vi "HOST_1712.vi"() -> ()   [LabVIEW 2018]
uses:
  <vilib>/userdefined/High Color/nirio_resource_hc.ctl
  <instrlib>/niDCPower/nidcpower.llb/niDCPower Measurement Type.ctl
  <vilib>/FPGAPlugInAG/PXI-7953R/niLvFpga_Open_PXI-7953R.vi
  <vilib>/rvi/interface/common/dynamic/niFpgaDynamicAddResources.vi
  <vilib>/FPGAPlugInAG/Dynamic/niLvFpga_Reset_Dynamic.vi
  <vilib>/FPGAPlugInAG/Dynamic/niLvFpga_Run_Dynamic.vi
  <vilib>/Utility/error.llb/Error Cluster From Error Code.vi
  <vilib>/rvi/errors/niLvFpgaAdjustHostInterfaceError.vi
  <vilib>/FPGAPlugInAG/Dynamic/niLvFpga_Close_Dynamic.vi
  <vilib>/rvi/interface/nirviOpenFPGA/nirviOpenFPGA.xnode
  FPGA Bitfiles/1712_FPGATarget_TARGET1712_pD+j9IKIark.lvbitx
  <vilib>/rvi/interface/nirviMethod/nirviMethod.xnode
  <vilib>/rvi/interface/nirviReadWriteControl/nirviReadWriteControl.xnode
  <vilib>/rvi/interface/nirviCloseFPGA/nirviCloseFPGA.xnode
  NiFpgaLv.dll
  <vilib>/rvi/interface/Simulation/niFpgaSimulationCallBeginRW.vi
  <vilib>/FPGAPlugInAG/Dynamic/niLvFpga_ReadFifo_Dynamic.vi
  <vilib>/rvi/errors/niLvFpgaMergeErrorWithErrorCode.vi
panel:
  in  "Tab Control":enum32{"Рабочая", "Служебная"}(tab)
  out "Image":T1(plugin-control)
  in  "Frames":path=path "D:/VPL/LabView/DOZOR_1712/DOZOR_1712/FRAMES"
  in  "LED":bool
  out "Номер образца":string="0"
  in  "Стоп":bool
  in  "Питание":bool
  in  "Линейки":bool
  in  "LOGS":path=path "D:/VPL/LabView/DOZOR_1712/DOZOR_1712/LOGS"
  in  "resource name":T2="PXI1Slot6"
  in  "1":refnum<k15>="PXI1Slot3" caption="instrument handle"
  in  "0":refnum<k15>="PXI1Slot2" caption="instrument handle"
  in  "2":refnum<k15>="PXI1Slot4" caption="instrument handle"
  in  "-15, V":dbl=-15.0 caption="voltage level" format="%_6p"
  out "-15_cur":dbl caption="measurement" format="%_6g"
  in  "-15_curlim":dbl=0.1 caption="current limit" format="%_6p"
  out "4V_cur":dbl caption="measurement" format="%_6g"
  in  "4V_curlim":dbl=0.15 caption="current limit" format="%_6p"
  in  "4V":dbl=4.0 caption="voltage level" format="%_6p"
  in  "1V":dbl=1.0 caption="voltage level" format="%_6p"
  in  "STAB, V":dbl=10.0 caption="voltage level" format="%_6p"
  out "VDD_cur":dbl caption="measurement" format="%_6g"
  out "1V_cur":dbl caption="measurement" format="%_6g"
  out "PH_LOW_cur":dbl caption="measurement" format="%_6g"
  out "RD_cur":dbl caption="measurement" format="%_6g"
  out "STAB_cur":dbl caption="measurement" format="%_6g"
  out "ADC_cur":dbl caption="measurement" format="%_6g"
  in  "VDD_curlim":dbl=0.15 caption="current limit" format="%_6p"
  in  "1V_curlim":dbl=0.01 caption="current limit" format="%_6p"
  in  "PH_LOW_curlim":dbl=0.3 caption="current limit" format="%_6p"
  in  "RD_curlim":dbl=0.1 caption="current limit" format="%_6p"
  in  "STAB_curlim":dbl=0.2 caption="current limit" format="%_6p"
  in  "ADC_curlim":dbl=0.2 caption="current limit" format="%_6p"
  in  "VDD, V":dbl=17.0 caption="voltage level" format="%_6p"
  in  "PH_LOW, V":dbl=-3.5 caption="voltage level" format="%_6p"
  in  "RD, V":dbl=13.1 caption="voltage level" format="%_6p"
  in  "ADC, V":dbl=6.0 caption="voltage level" format="%_6p"
  out "PS_LOW_cur":dbl caption="measurement" format="%_6g"
  in  "PS_LOW_curlim":dbl=0.1 caption="current limit" format="%_6p"
  in  "PS_LOW, V":dbl=-8.0 caption="voltage level" format="%_6p"
  out "ADC":bool
  out "4V":bool
  out "1V":bool
  out "1V":i32
  out "PH":i32
  out "RD":i32
  out "4V":i32
  out "-15":i32
  out "STAB":i32
  out "ADC":i32
  out "PS":i32
  out "VDD":i32
  in  "4V_selcur":dbl=0.025 caption="current limit" format="%_6p"
  in  "RD_selcur":dbl=0.01 caption="current limit" format="%_6p"
  in  "PH_LOW_selcur":dbl=0.025 caption="current limit" format="%_6p"
  in  "ADC_selcur":dbl=0.15 caption="current limit" format="%_6p"
  in  "STAB_selcur":dbl=0.1 caption="current limit" format="%_6p"
  in  "-15_selcur":dbl=0.009999999999999998 caption="current limit" format="%_6p"
  in  "1V_selcur":dbl=0.01 caption="current limit" format="%_6p"
  in  "VDD_selcur":dbl=0.075 caption="current limit" format="%_6p"
  in  "PS_LOW_selcur":dbl=0.01 caption="current limit" format="%_6p"
  out "STAB":bool
  out "-15":bool
  out "RD":bool
  out "PH":bool
  out "VDD":bool
  out "PS":bool
  in  "Какая фотка?":string
  in  "ПРИМЕЧАНИЕ":string
  out "СКО":dbl
  out "Среднее":dbl
  in  "Запись Кадра":bool
  out "FRAME_OK":bool
  in  "2/4 V":enum16{"2V", "4V"}(ring)
  in  "3CH/1CH":enum16{"3CH", "1CH"}(ring)=enum."1CH"
  out "Configuration":bool[](array[boolean])
  in  "Какой канал?":enum16{"OUT1", "OUT2", "OUT3"}(ring)
  in  "Прошить АЦП":bool
  out "АЦП прошит!":bool
  in  "НЕПРЕРЫВНО":bool
  in  "文韧 世男!":bool
  in  "ПЕРЕБОР?":bool
  out "Канал":string="1"
  in  "SIM_SEL":bool
  out "SEL":bool
  out "FRAME":u16[][](array[numeric])
  out "OUT":cluster{u16, u16, u16, u16}[][](array[cluster])
  in  "Сколько строк?":i32=270
  in  "1163":u16=1163
  in  "PS1_2":u16=980
  in  "PS1_1":u16=300
  in  "PS21_1":u16=165
  in  "PS21_2":u16=573
  in  "PS3_1":u16=435
  in  "PS3_2":u16=843
  in  "PS41_1":u16=30
  in  "PS41_2":u16=710
  in  "CDS1_2":u8=14
  in  "CDS1_1":u8=9
  in  "CDS2_2":u8=18
  in  "CDS2_1":u8=5
  in  "ADC_2":u8=22
  in  "ADC_1":u8=9
  in  "RG_2":u8=8
  in  "RG1":u8=5
  in  "PH2_2":u8=17
  in  "PH2_1":u8=5
  in  "PH1_2":u8=17
  in  "PH1_1":u8=5
  in  "HOR":u16=465
  in  "8":u8=24
  in  "LOW":u8=9
  in  "HIGH":u8=22
  in  "Усреднение":i32=1
  in  "Между кадрами, мс":u8=1
  in  "ISO":dbl=1.0
  in  "+/- OUT2":enum16{"-", "+"}(ring)=enum."+"
  in  "Смещение, до 300_OUT2":dbl
  in  "Усиление (до 6)_OUT2":u8=1
  in  "Усиление (до 6)_OUT4":u8=1
  in  "+/- OUT4":enum16{"-", "+"}(ring)=enum."+"
  in  "Смещение, до 300_OUT4":dbl
  in  "Усиление (до 6)_OUT1":u8=1
  in  "Смещение, до 300_OUT1":dbl
  in  "+/- OUT1":enum16{"-", "+"}(ring)=enum."+"
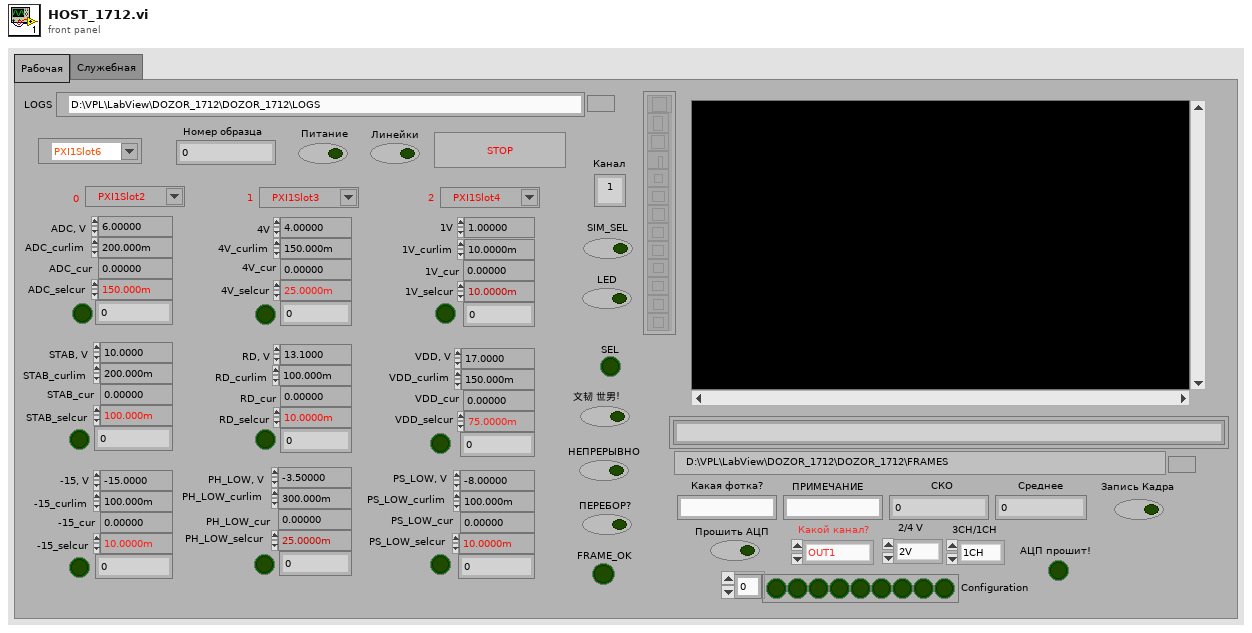
[diagram p1: front panel]
types:
  T1 = typedef "IMAQ Image.ctl" = refnum<image>
  T2 = typedef "nirio_resource_hc.ctl" = tag
  T3 = enum16{"open", "replace", "create", "open or create", "replace or create", "replace or create with confirmation"}
  T4 = typedef "niDCPower Measurement Type.ctl" = i32
  T5 = typedef "Image Type" = u32
  T6 = enum16{"Configuration", "MUX", "RED PGA", "GREEN PGA", "BLUE PGA", "RED OFF", "GREEN OFF", "BLUE OFF"}
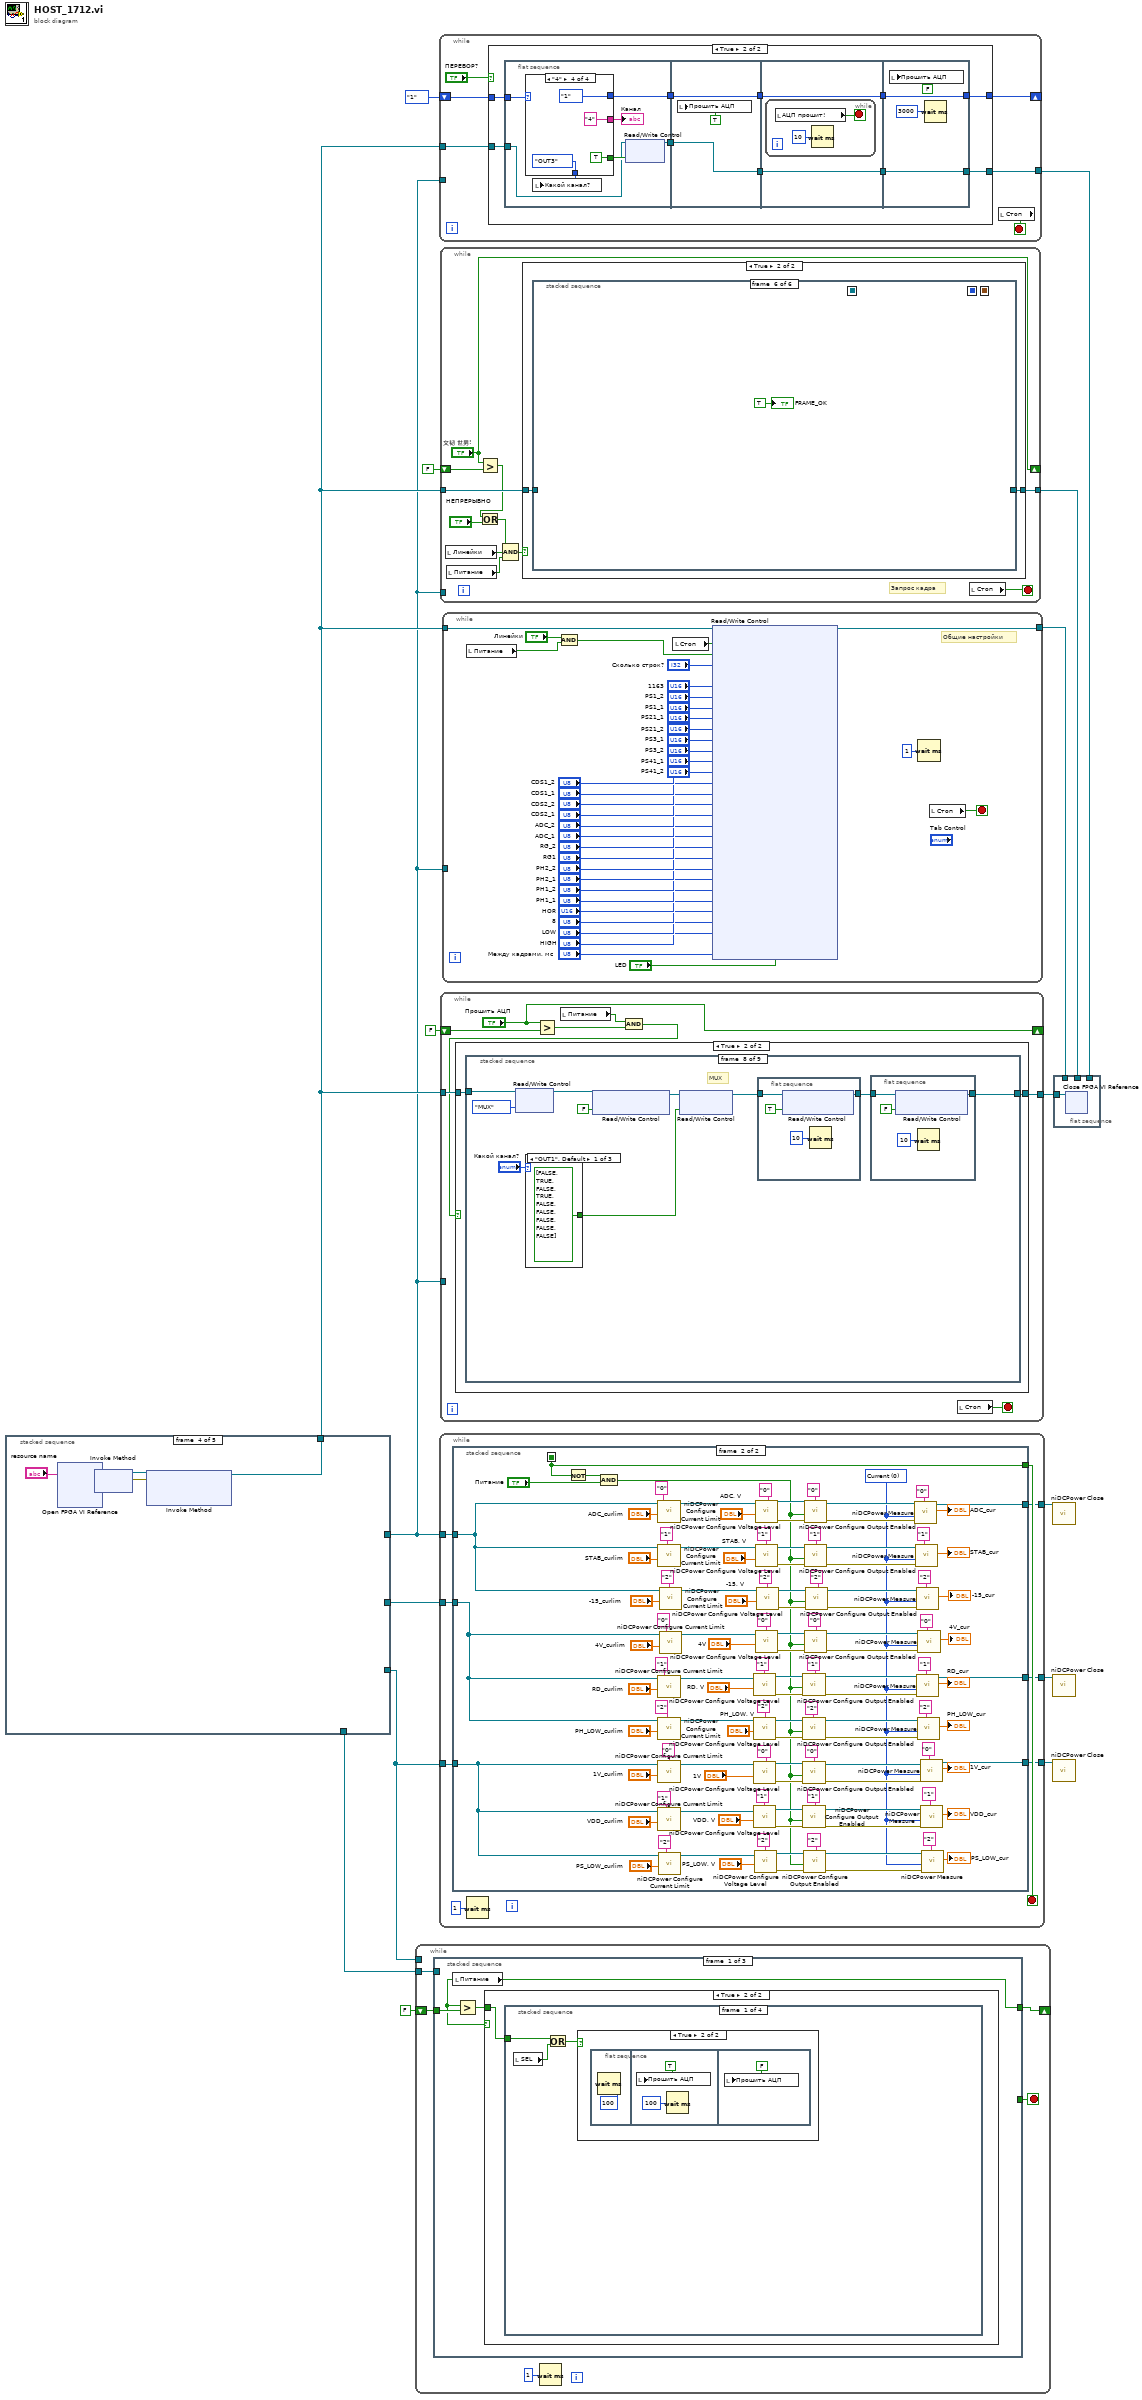
[diagram p0: block diagram]
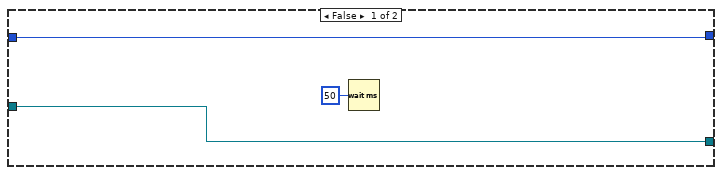
[diagram p2: hidden frame]
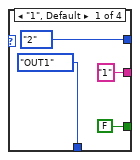
[diagram p3: hidden frame]
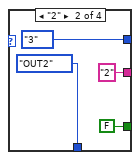
[diagram p4: hidden frame]
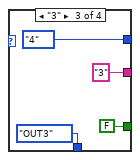
[diagram p5: hidden frame]
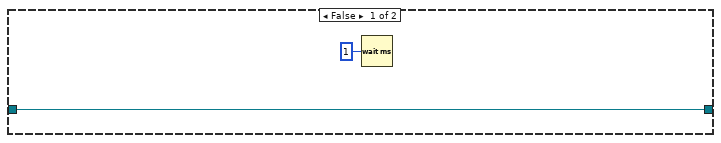
[diagram p6: hidden frame]
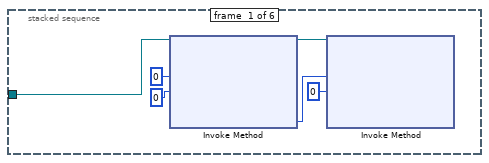
[diagram p7: hidden frame]
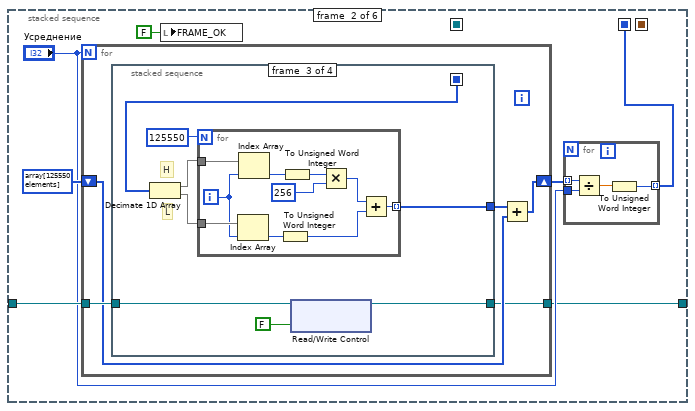
[diagram p8: hidden frame]
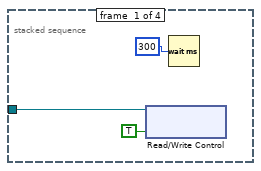
[diagram p9: hidden frame]
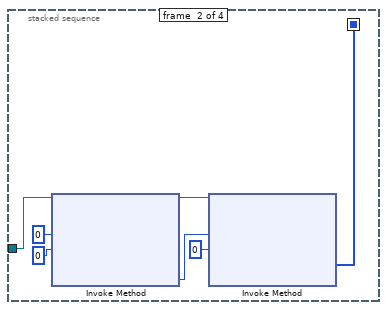
[diagram p10: hidden frame]
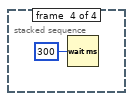
[diagram p11: hidden frame]
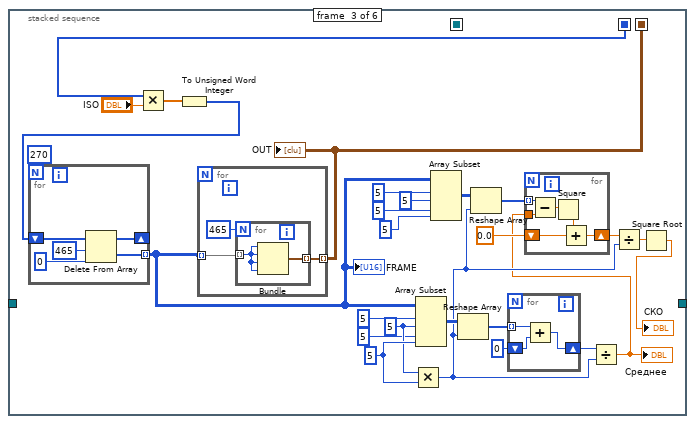
[diagram p12: hidden frame]
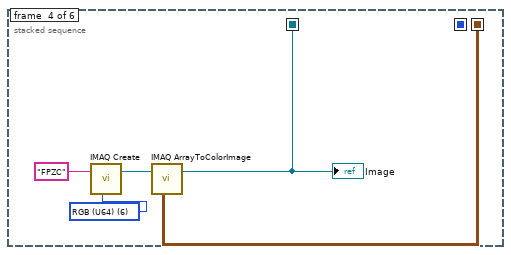
[diagram p13: hidden frame]
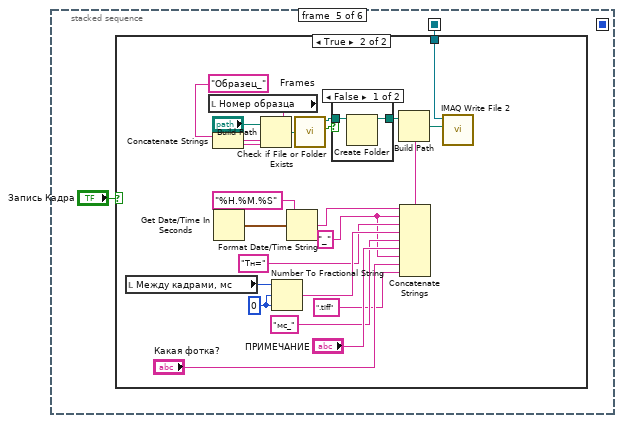
[diagram p14: hidden frame]
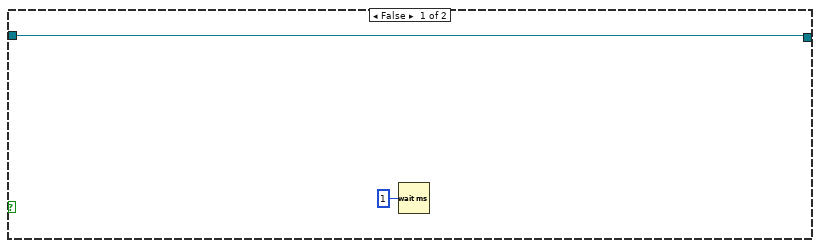
[diagram p17: hidden frame]
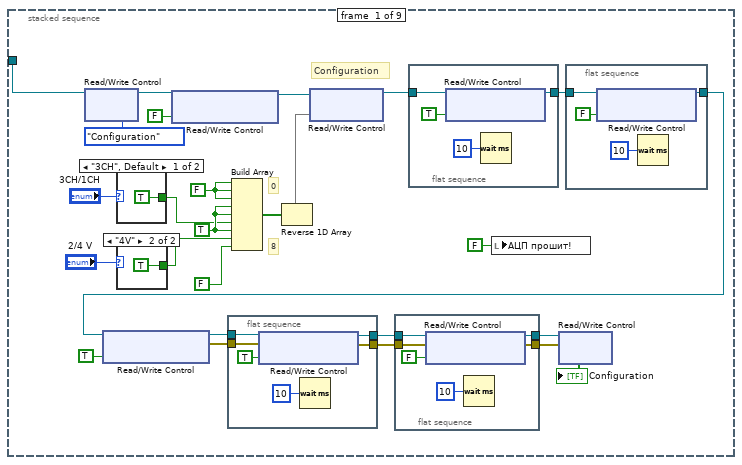
[diagram p18: hidden frame]
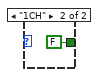
[diagram p19: hidden frame]
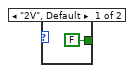
[diagram p20: hidden frame]
diagram:
  n1 = stacked-sequence {
    tunnel: [_ _ _ _ w67] -> w6
    tunnel: [_ _ _ _ w66] -> w9
    tunnel: [_ _ _ _ w65] -> w16
    tunnel: [_ _ _ w59 _] -> w10
    tunnel: [_ _ w22 _ _] -> w11
    frame #0 {
      n2 = call "Begin.vi"() -> ("Номер образца 2"=→"Номер образца":string)  [unwired: 11 in]
    }
    frame #1 {
      w18 = FALSE
      w20 = 0 ("VDD")
      w19 = "" ("Какая фотка?")
      # "Отжатие кнопок, обнуление счетчиков"
      n3 = local write "Какой канал?"(enum16{"OUT1", "OUT2", "OUT3"}."OUT1" ("Какой канал?")) -> ()
      n4 = local write "Запись Кадра"(w18) -> ()
      n5 = local write "НЕПРЕРЫВНО"(w18) -> ()
      n6 = local write "ПЕРЕБОР?"(w18) -> ()
      n7 = local write "FRAME_OK"(w18) -> ()
      n8 = local write "Прошить АЦП"(w18) -> ()
      n9 = local write "文韧 世男!"(w18) -> ()
      n10 = local write "АЦП прошит!"(w18) -> ()
      n11 = local write "SIM_SEL"(w18) -> ()
      n12 = local write "Стоп"(w18) -> ()
      n13 = local write "Питание"(w18) -> ()
      n14 = local write "Линейки"(w18) -> ()
      n15 = local write "LED"(w18) -> ()
      n16 = local write "Какая фотка?"(w19) -> ()
      n17 = local write "ПРИМЕЧАНИЕ"(w19) -> ()
      n18 = local write "VDD"(w20) -> ()
      n19 = local write "RD"(w20) -> ()
      n20 = local write "PH"(w20) -> ()
      n21 = local write "PS"(w20) -> ()
      n22 = local write "1V"(w20) -> ()
      n23 = local write "ADC"(w20) -> ()
      n24 = local write "STAB"(w20) -> ()
      n25 = local write "-15"(w20) -> ()
      n26 = local write "4V"(w20) -> ()
    }
    frame #2 {
      w24 = "\t"
      n27 = local read "Номер образца"() -> (w51:string)
      n28 = Build Path(base path="LOGS", name or relative path=w51) -> (appended path=w48:path)
      n29 = Get Date/Time In Seconds() -> (seconds since 1Jan1904=w45:timestamp)
      n30 = call <vilib>:"Check if File or Folder Exists.vi"("path"=w48) -> ("file or folder exists?"=w49:bool, "dup path"=w50:path)  [unwired: 8 in, 1 out]
      n31 = Format Date/Time String(time format string (%c)="%d %H.%M.%S", seconds (now)=w45) -> (date/time string=w43:string)  [unwired: 1 in]
      n32 = case shown="False" w49 {
        tunnel: w50 -> [w57 w58]
        tunnel: [w56 w58] -> w40
        frame False {
          n33 = Create Folder(path (use dialog)=w57) -> (created path=w56:path)  [unwired: 2 in, 2 out]
        }
        frame True {
        }
      }
      n34 = Concatenate Strings(w43, ".xls" ("string")) -> (w42:string)
      n35 = Build Path(base path=w40, name or relative path=w42) -> (appended path=w44:path)
      n36 = Open/Create/Replace File(file path (use dialog)=w44, operation (0:open)=T3."open or create", access (0:read/write)=enum16{"read/write", "read-only", "write-only"}."read/write") -> (refnum out=w46:refnum<file>)  [unwired: 3 in, 2 out]
      n37 = case shown="True" TRUE {
        tunnel: w46 -> [w52 w55]
        tunnel: [w52 w53] -> w41
        frame False {
        }
        frame True {
          n38 = Set File Position(refnum=w55, from (0:start)=enum16{"start", "end", "current"}."end") -> (refnum out=w53:refnum<file>)  [unwired: 2 in, 1 out]
        }
      }
      n39 = Format Into String(initial string=w41, "Time" ("input 1"), w24, "ADC_cur", w24, "STAB_cur", w24, "-15_cur", w24, "4_cur", w24, "RD_cur", w24, "PH_LOW_cur", w24, "1V_cur", w24, "VDD_cur", w24, "PS_LOW_cur", "\r\n") -> (resulting string=w22:refnum<file>)  [unwired: 2 in, 1 out]
    }
    frame #3 {
      n40 = xnode "Open FPGA VI Reference"("resource name"="resource name") -> ("FPGA VI Reference Out"=w60:refnum<k20>, "error out"=w62:errorcluster)  [unwired: 1 in]
      n41 = xnode "Invoke Method"("FPGA VI Reference In"=w60, "error in"=w62) -> ("FPGA VI Reference Out"=w63:refnum<k20>, "error out"=w61:errorcluster)
      n42 = xnode "Invoke Method"("FPGA VI Reference In"=w63, "error in"=w61) -> ("FPGA VI Reference Out"=w59:refnum<k20>)  [unwired: 1 in, 1 out]
    }
    frame #4 {
      n43 = call <instrlib>:"niDCPower Initialize.vi"("resource name"="2") -> ("error out"=w73:errorcluster, "instrument handle out"=w70:refnum<k15>)  [unwired: 3 in, 6 out]
      n44 = call <instrlib>:"niDCPower Initialize.vi"("resource name"="1") -> ("error out"=w71:errorcluster, "instrument handle out"=w68:refnum<k15>)  [unwired: 3 in, 6 out]
      n45 = call <instrlib>:"niDCPower Initialize.vi"("resource name"="0") -> ("error out"=w72:errorcluster, "instrument handle out"=w69:refnum<k15>)  [unwired: 3 in, 6 out]
      n46 = call <instrlib>:"niDCPower Configure Voltage Level.vi"("error in (no error)"=w73, "voltage level"=0.0, "channel name"="0,1,2", "instrument handle"=w70) -> ("instrument handle out"=w67:refnum<k15>)  [unwired: 6 in, 1 out]
      n47 = call <instrlib>:"niDCPower Configure Voltage Level.vi"("error in (no error)"=w71, "voltage level"=0.0, "channel name"="0,1,2", "instrument handle"=w68) -> ("instrument handle out"=w65:refnum<k15>)  [unwired: 6 in, 1 out]
      n48 = call <instrlib>:"niDCPower Configure Voltage Level.vi"("error in (no error)"=w72, "voltage level"=0.0, "channel name"="0,1,2", "instrument handle"=w69) -> ("instrument handle out"=w66:refnum<k15>)  [unwired: 6 in, 1 out]
    }
  }
  n49 = while {
    tunnel: w11 -> [w85]
    shift-right: [w83] -> _
    shift-left: FALSE -> [w84]
    tunnel: w6 -> [_]
    stop <- w86 stop-if-true
    n50 = stacked-sequence {
      tunnel: [_ _ w227] -> w86
      tunnel: w85 -> [_ w203 _]
      tunnel: w84 -> [w90 _ _]
      tunnel: [w88 _ _] -> w83
      frame #0 {
        n51 = local read "Питание"() -> (w88:bool)
        n52 = Greater?(x=w88, y=w90) -> (0:w89:bool)
        n53 = case shown="True" w88 {
          tunnel: w89 -> [_ w91]
          frame False {
          }
          frame True {
            n54 = stacked-sequence {
              tunnel: w91 -> [w93 _ _ _]
              frame #0 {
                n55 = local read "SEL"() -> (w92:bool)
                n56 = Or(x=w93, y=w92) -> (x .or. y?=w94:bool)
                n57 = case shown="True" w94 {
                  frame False {
                  }
                  frame True {
                    n58 = flat-sequence {
                      frame #0 {
                        n59 = Wait (ms)(milliseconds to wait=u32 100) -> ()  [unwired: 1 out]
                      }
                      frame #1 {
                        n60 = local write "Прошить АЦП"(TRUE ("Прошить АЦП")) -> ()
                        n61 = Wait (ms)(milliseconds to wait=u32 100) -> ()  [unwired: 1 out]
                      }
                      frame #2 {
                        n62 = local write "Прошить АЦП"(FALSE ("Прошить АЦП")) -> ()
                      }
                    }
                  }
                }
              }
              frame #1 {
                n63 = local read "PH_LOW_cur"() -> (w121:dbl)
                n64 = local read "PS_LOW_cur"() -> (w124:dbl)
                n65 = local read "STAB_cur"() -> (w100:dbl)
                n66 = local read "ADC_cur"() -> (w109:dbl)
                n67 = local read "VDD_cur"() -> (w106:dbl)
                n68 = local read "-15_cur"() -> (w118:dbl)
                n69 = local read "RD_cur"() -> (w103:dbl)
                n70 = local read "4V_cur"() -> (w112:dbl)
                n71 = local read "1V_cur"() -> (w115:dbl)
                n72 = Greater?(x=w100, y="STAB_selcur") -> (0:→"STAB":bool)
                n73 = Greater?(x=w103, y="RD_selcur") -> (0:→"RD":bool)
                n74 = Greater?(x=w106, y="VDD_selcur") -> (0:→"VDD":bool)
                n75 = Greater?(x=w109, y="ADC_selcur") -> (0:→"ADC":bool)
                n76 = Greater?(x=w112, y="4V_selcur") -> (0:→"4V":bool)
                n77 = Greater?(x=w115, y="1V_selcur") -> (0:→"1V":bool)
                n78 = Greater?(x=w118, y="-15_selcur") -> (0:→"-15":bool)
                n79 = Greater?(x=w121, y="PH_LOW_selcur") -> (0:→"PH":bool)
                n80 = Greater?(x=w124, y="PS_LOW_selcur") -> (0:→"PS":bool)
              }
              frame #2 {
                n81 = local read "ADC"() -> (w132:bool)
                n82 = local read "STAB"() -> (w133:bool)
                n83 = local read "-15"() -> (w134:bool)
                n84 = local read "4V"() -> (w129:bool)
                n85 = local read "VDD"() -> (w130:bool)
                n86 = local read "PS"() -> (w131:bool)
                n87 = case shown="True" w130 {
                  frame False {
                  }
                  frame True {
                    n88 = local read "VDD"() -> (w152:i32)
                    n89 = Increment(x=w152) -> (x+1=→"VDD":i32)
                  }
                }
                n90 = case shown="True" w131 {
                  frame False {
                  }
                  frame True {
                    n91 = local read "PS"() -> (w150:i32)
                    n92 = Increment(x=w150) -> (x+1=→"PS":i32)
                  }
                }
                n93 = case shown="True" w132 {
                  frame False {
                  }
                  frame True {
                    n94 = local read "ADC"() -> (w148:i32)
                    n95 = Increment(x=w148) -> (x+1=→"ADC":i32)
                  }
                }
                n96 = case shown="True" w133 {
                  frame False {
                  }
                  frame True {
                    n97 = local read "STAB"() -> (w146:i32)
                    n98 = Increment(x=w146) -> (x+1=→"STAB":i32)
                  }
                }
                n99 = case shown="True" w134 {
                  frame False {
                  }
                  frame True {
                    n100 = local read "-15"() -> (w144:i32)
                    n101 = Increment(x=w144) -> (x+1=→"-15":i32)
                  }
                }
                n102 = case shown="True" w129 {
                  frame False {
                  }
                  frame True {
                    n103 = local read "4V"() -> (w142:i32)
                    n104 = Increment(x=w142) -> (x+1=→"4V":i32)
                  }
                }
                n105 = local read "RD"() -> (w128:bool)
                n106 = local read "PH"() -> (w127:bool)
                n107 = local read "1V"() -> (w126:bool)
                n108 = case shown="True" w127 {
                  frame False {
                  }
                  frame True {
                    n109 = local read "PH"() -> (w138:i32)
                    n110 = Increment(x=w138) -> (x+1=→"PH":i32)
                  }
                }
                n111 = case shown="True" w128 {
                  frame False {
                  }
                  frame True {
                    n112 = local read "RD"() -> (w140:i32)
                    n113 = Increment(x=w140) -> (x+1=→"RD":i32)
                  }
                }
                n114 = case shown="True" w126 {
                  frame False {
                  }
                  frame True {
                    n115 = local read "1V"() -> (w136:i32)
                    n116 = Increment(x=w136) -> (x+1=→"1V":i32)
                  }
                }
              }
              frame #3 {
                n117 = local read "STAB"() -> (w163:bool)
                n118 = local read "ADC"() -> (w164:bool)
                n119 = local read "VDD"() -> (w166:bool)
                n120 = local read "-15"() -> (w162:bool)
                n121 = local read "PH"() -> (w159:bool)
                n122 = local read "RD"() -> (w160:bool)
                n123 = local read "PS"() -> (w165:bool)
                n124 = local read "4V"() -> (w161:bool)
                n125 = local read "1V"() -> (w158:bool)
                n126 = Compound Arithmetic op=OR(w166, w165, w164, w163, w162, w161, w160, w159, w158) -> (w154:bool)
                n127 = local read "Линейки"() -> (w156:bool)
                n128 = local read "Питание"() -> (w157:bool)
                n129 = Or(x=w154, y="SIM_SEL") -> (x .or. y?=w153:bool)
                "SEL" <- w153
                n130 = case shown="True" w153 {
                  tunnel: w156 -> [_ w173]
                  tunnel: w157 -> [_ w172]
                  frame False {
                    n131 = Wait (ms)(milliseconds to wait=u32 1) -> ()  [unwired: 1 out]
                  }
                  frame True {
                    n132 = flat-sequence {
                      tunnel: w173 -> [w175]
                      tunnel: w172 -> [w174]
                      tunnel: [w175] -> w170
                      tunnel: [w174] -> w169
                      tunnel: [w178] -> w171
                      tunnel: w170 -> [w178]
                      tunnel: w169 -> [w177]
                      tunnel: [w177] -> w168
                      tunnel: w171 -> [w181]
                      tunnel: w168 -> [w180]
                      frame #0 {
                        w176 = FALSE ("Питание")
                        n133 = local write "Питание"(w176) -> ()
                        n134 = local write "Линейки"(w176) -> ()
                      }
                      frame #1 {
                        n135 = Wait (ms)(milliseconds to wait=u32 100) -> ()  [unwired: 1 out]
                      }
                      frame #2 {
                        n136 = local write "Линейки"(w181) -> ()
                        n137 = local write "Питание"(w180) -> ()
                      }
                    }
                  }
                }
              }
            }
          }
        }
      }
      frame #1 {
        w202 = i16 0 ("width (-)")
        w205 = i16 3 ("width (-)")
        w201 = "\t"
        # "Логирование данных"
        n138 = local read "STAB"() -> (w189:i32)
        n139 = local read "ADC"() -> (w190:i32)
        n140 = local read "VDD"() -> (w183:i32)
        n141 = local read "-15"() -> (w188:i32)
        n142 = local read "PH"() -> (w185:i32)
        n143 = local read "RD"() -> (w186:i32)
        n144 = local read "4V"() -> (w187:i32)
        n145 = local read "1V"() -> (w184:i32)
        n146 = local read "PS"() -> (w182:i32)
        n147 = Number To Fractional String(number=w190, width (-)=w202, precision (6)=w202) -> (F-format string=w199:string)  [unwired: 1 in]
        n148 = Number To Fractional String(number=w189, width (-)=w202, precision (6)=w202) -> (F-format string=w198:string)  [unwired: 1 in]
        n149 = Number To Fractional String(number=w188, width (-)=w202, precision (6)=w202) -> (F-format string=w197:string)  [unwired: 1 in]
        n150 = Number To Fractional String(number=w187, width (-)=w202, precision (6)=w202) -> (F-format string=w196:string)  [unwired: 1 in]
        n151 = Number To Fractional String(number=w186, width (-)=w202, precision (6)=w202) -> (F-format string=w195:string)  [unwired: 1 in]
        n152 = Number To Fractional String(number=w185, width (-)=w202, precision (6)=w202) -> (F-format string=w194:string)  [unwired: 1 in]
        n153 = Number To Fractional String(number=w184, width (-)=w202, precision (6)=w202) -> (F-format string=w193:string)  [unwired: 1 in]
        n154 = Number To Fractional String(number=w183, width (-)=w202, precision (6)=w202) -> (F-format string=w192:string)  [unwired: 1 in]
        n155 = Number To Fractional String(number=w182, width (-)=w202, precision (6)=w202) -> (F-format string=w191:string)  [unwired: 1 in]
        n156 = local read "PH_LOW_cur"() -> (w209:dbl)
        n157 = local read "PS_LOW_cur"() -> (w206:dbl)
        n158 = local read "STAB_cur"() -> (w213:dbl)
        n159 = local read "ADC_cur"() -> (w214:dbl)
        n160 = local read "VDD_cur"() -> (w207:dbl)
        n161 = local read "-15_cur"() -> (w212:dbl)
        n162 = local read "RD_cur"() -> (w210:dbl)
        n163 = local read "4V_cur"() -> (w211:dbl)
        n164 = local read "1V_cur"() -> (w208:dbl)
        n165 = Number To Fractional String(number=w214, width (-)=w205, precision (6)=w205) -> (F-format string=w223:string)  [unwired: 1 in]
        n166 = Number To Fractional String(number=w213, width (-)=w205, precision (6)=w205) -> (F-format string=w222:string)  [unwired: 1 in]
        n167 = Number To Fractional String(number=w212, width (-)=w205, precision (6)=w205) -> (F-format string=w221:string)  [unwired: 1 in]
        n168 = Number To Fractional String(number=w211, width (-)=w205, precision (6)=w205) -> (F-format string=w220:string)  [unwired: 1 in]
        n169 = Number To Fractional String(number=w210, width (-)=w205, precision (6)=w205) -> (F-format string=w219:string)  [unwired: 1 in]
        n170 = Number To Fractional String(number=w209, width (-)=w205, precision (6)=w205) -> (F-format string=w218:string)  [unwired: 1 in]
        n171 = Number To Fractional String(number=w208, width (-)=w205, precision (6)=w205) -> (F-format string=w217:string)  [unwired: 1 in]
        n172 = Number To Fractional String(number=w207, width (-)=w205, precision (6)=w205) -> (F-format string=w216:string)  [unwired: 1 in]
        n173 = Number To Fractional String(number=w206, width (-)=w205, precision (6)=w205) -> (F-format string=w215:string)  [unwired: 1 in]
        n174 = Get Date/Time In Seconds() -> (seconds since 1Jan1904=w226:timestamp)
        n175 = Format Date/Time String(time format string (%c)="%d %H:%M:%S:%3u", seconds (now)=w226) -> (date/time string=w224:string)  [unwired: 1 in]
        n176 = Concatenate Strings(w224, w201, w223, w201, w222, w201, w221, w201, w220, w201, w219, w201, w218, w201, w217, w201, w216, w201, w215, w201, w199, w201, w198, w201, w197, w201, w196, w201, w195, w201, w194, w201, w193, w201, w192, w201, w191, "\r\n") -> (w225:string)
        n177 = Format Into String(initial string=w203, w225) -> ()  [unwired: 2 in, 2 out]
      }
      frame #2 {
        n178 = local read "Стоп"() -> (w227:bool)
      }
    }
    n179 = Wait (ms)(milliseconds to wait=u32 1) -> ()  [unwired: 1 out]
  }
  n180 = while {
    tunnel: w10 -> [w231]
    tunnel: w9 -> [_]
    shift-right: [w229] -> _
    shift-left: enum16{"1", "2", "3", "4"}."1" -> [w230]
    tunnel: [w228] -> w1
    stop <- w233 stop-if-true
    n181 = case shown="True" "ПЕРЕБОР?" {
      tunnel: w231 -> [w234 w246]
      tunnel: w230 -> [w235 w245]
      tunnel: [w235 w241] -> w229
      tunnel: [w234 w240] -> w228
      frame False {
        n182 = Wait (ms)(milliseconds to wait=u32 50) -> ()  [unwired: 1 out]
      }
      frame True {
        n183 = flat-sequence {
          tunnel: w246 -> [w249]
          tunnel: w245 -> [w253]
          tunnel: [w252] -> w244
          tunnel: [w247] -> w237
          tunnel: w244 -> [w271]
          tunnel: [w271] -> w242
          tunnel: [w270] -> w238
          tunnel: w237 -> [w270]
          tunnel: [w274] -> w243
          tunnel: w242 -> [w274]
          tunnel: [w273] -> w239
          tunnel: w238 -> [w273]
          tunnel: w243 -> [w278]
          tunnel: [w278] -> w241
          tunnel: [w277] -> w240
          tunnel: w239 -> [w277]
          frame #0 {
            n184 = case shown="\"4\"" w253 {
              tunnel: [enum16{"1", "2", "3", "4"}."2" enum16{"1", "2", "3", "4"}."3" enum16{"1", "2", "3", "4"}."4" enum16{"1", "2", "3", "4"}."1"] -> w252
              tunnel: [FALSE ("VNR") FALSE ("VNR") FALSE ("VNR") TRUE ("VNR")] -> w251
              tunnel: ["1" "2" "3" "4"] -> w250
              tunnel: [enum16{"OUT1", "OUT2", "OUT3"}."OUT1" ("Какой канал?") enum16{"OUT1", "OUT2", "OUT3"}."OUT2" ("Какой канал?") enum16{"OUT1", "OUT2", "OUT3"}."OUT3" ("Какой канал?") enum16{"OUT1", "OUT2", "OUT3"}."OUT3" ("Какой канал?")] -> w248
              frame "1", Default {
              }
              frame "2" {
              }
              frame "3" {
              }
              frame "4" {
              }
            }
            "Канал" <- w250
            n185 = local write "Какой канал?"(w248) -> ()
            n186 = xnode "Read/Write Control"("FPGA VI Reference In"=w249, "VNR"=w251) -> ("FPGA VI Reference Out"=w247:refnum<k20>)  [unwired: 1 in, 1 out]
          }
          frame #1 {
            n187 = local write "Прошить АЦП"(TRUE ("Прошить АЦП")) -> ()
          }
          frame #2 {
            n188 = while {
              stop <- w276 stop-if-true
              n189 = local read "АЦП прошит!"() -> (w276:bool)
              n190 = Wait (ms)(milliseconds to wait=u32 10) -> ()  [unwired: 1 out]
            }
          }
          frame #3 {
            n191 = local write "Прошить АЦП"(FALSE ("Прошить АЦП")) -> ()
            n192 = Wait (ms)(milliseconds to wait=u32 3000) -> ()  [unwired: 1 out]
          }
        }
      }
    }
    n193 = local read "Стоп"() -> (w233:bool)
  }
  n194 = while {
    tunnel: w9 -> [w287]
    tunnel: w16 -> [w286]
    tunnel: w6 -> [w285]
    tunnel: [w283] -> w15
    tunnel: [w282] -> w14
    tunnel: [w281] -> w13
    stop <- w284 stop-if-true
    n195 = stacked-sequence {
      seq-local: ["Стоп" _] -> [_ w290]
      tunnel: w285 -> [_ w295]
      tunnel: [_ w336] -> w283
      tunnel: [_ w335] -> w282
      tunnel: [_ w334] -> w281
      tunnel: w287 -> [_ w294]
      tunnel: w286 -> [_ w293]
      tunnel: [_ w290] -> w284
      frame #0 {
      }
      frame #1 {
        w296 = T4 0 items=["Current", "Voltage"] ("measurement type")
        n196 = Not(x=w290) -> (.not. x?=w309:bool)
        n197 = And(x=w309, y="Питание") -> (x .and. y?=w291:bool)
        n198 = call <instrlib>:"niDCPower Configure Current Limit.vi"("current limit"="ADC_curlim", "channel name"="0", "instrument handle"=w294) -> ("instrument handle out"=w371:refnum<k15>)  [unwired: 7 in, 1 out]
        n199 = call <instrlib>:"niDCPower Configure Current Limit.vi"("current limit"="STAB_curlim", "channel name"="1", "instrument handle"=w294) -> ("instrument handle out"=w372:refnum<k15>)  [unwired: 7 in, 1 out]
        n200 = call <instrlib>:"niDCPower Configure Current Limit.vi"("current limit"="RD_curlim", "channel name"="1", "instrument handle"=w293) -> ("instrument handle out"=w373:refnum<k15>)  [unwired: 7 in, 1 out]
        n201 = call <instrlib>:"niDCPower Configure Current Limit.vi"("current limit"="PH_LOW_curlim", "channel name"="2", "instrument handle"=w293) -> ("instrument handle out"=w374:refnum<k15>)  [unwired: 7 in, 1 out]
        n202 = call <instrlib>:"niDCPower Configure Current Limit.vi"("current limit"="1V_curlim", "channel name"="0", "instrument handle"=w295) -> ("instrument handle out"=w375:refnum<k15>)  [unwired: 7 in, 1 out]
        n203 = call <instrlib>:"niDCPower Configure Current Limit.vi"("current limit"="VDD_curlim", "channel name"="1", "instrument handle"=w295) -> ("instrument handle out"=w376:refnum<k15>)  [unwired: 7 in, 1 out]
        n204 = call <instrlib>:"niDCPower Configure Current Limit.vi"("current limit"="PS_LOW_curlim", "channel name"="2", "instrument handle"=w295) -> ("instrument handle out"=w302:refnum<k15>)  [unwired: 7 in, 1 out]
        n205 = call <instrlib>:"niDCPower Configure Current Limit.vi"("current limit"="-15_curlim", "channel name"="2", "instrument handle"=w294) -> ("instrument handle out"=w316:refnum<k15>)  [unwired: 7 in, 1 out]
        n206 = call <instrlib>:"niDCPower Configure Current Limit.vi"("current limit"="4V_curlim", "channel name"="0", "instrument handle"=w293) -> ("instrument handle out"=w327:refnum<k15>)  [unwired: 7 in, 1 out]
        n207 = call <instrlib>:"niDCPower Configure Voltage Level.vi"("voltage level"="RD, V", "channel name"="1", "instrument handle"=w373) -> ("error out"=w354:errorcluster, "instrument handle out"=w351:refnum<k15>)  [unwired: 7 in]
        n208 = call <instrlib>:"niDCPower Configure Voltage Level.vi"("voltage level"="PH_LOW, V", "channel name"="2", "instrument handle"=w374) -> ("error out"=w353:errorcluster, "instrument handle out"=w352:refnum<k15>)  [unwired: 7 in]
        n209 = call <instrlib>:"niDCPower Configure Voltage Level.vi"("voltage level"="1V", "channel name"="0", "instrument handle"=w375) -> ("error out"=w363:errorcluster, "instrument handle out"=w366:refnum<k15>)  [unwired: 7 in]
        n210 = call <instrlib>:"niDCPower Configure Voltage Level.vi"("voltage level"="VDD, V", "channel name"="1", "instrument handle"=w376) -> ("error out"=w364:errorcluster, "instrument handle out"=w365:refnum<k15>)  [unwired: 7 in]
        n211 = call <instrlib>:"niDCPower Configure Voltage Level.vi"("voltage level"="PS_LOW, V", "channel name"="2", "instrument handle"=w302) -> ("error out"=w305:errorcluster, "instrument handle out"=w304:refnum<k15>)  [unwired: 7 in]
        n212 = call <instrlib>:"niDCPower Configure Voltage Level.vi"("voltage level"="ADC, V", "channel name"="0", "instrument handle"=w371) -> ("error out"=w341:errorcluster, "instrument handle out"=w344:refnum<k15>)  [unwired: 7 in]
        n213 = call <instrlib>:"niDCPower Configure Voltage Level.vi"("voltage level"="STAB, V", "channel name"="1", "instrument handle"=w372) -> ("error out"=w342:errorcluster, "instrument handle out"=w343:refnum<k15>)  [unwired: 7 in]
        n214 = call <instrlib>:"niDCPower Configure Voltage Level.vi"("voltage level"="4V", "channel name"="0", "instrument handle"=w327) -> ("error out"=w331:errorcluster, "instrument handle out"=w332:refnum<k15>)  [unwired: 7 in]
        n215 = call <instrlib>:"niDCPower Configure Voltage Level.vi"("voltage level"="-15, V", "channel name"="2", "instrument handle"=w316) -> ("error out"=w319:errorcluster, "instrument handle out"=w318:refnum<k15>)  [unwired: 7 in]
        n216 = call <instrlib>:"niDCPower Configure Output Enabled.vi"("error in (no error)"=w354, "output enabled"=w291, "channel name"="1", "instrument handle"=w351) -> ("error out"=w400:errorcluster, "instrument handle out"=w393:refnum<k15>)  [unwired: 6 in]
        n217 = call <instrlib>:"niDCPower Configure Output Enabled.vi"("error in (no error)"=w353, "output enabled"=w291, "channel name"="2", "instrument handle"=w352) -> ("error out"=w395:errorcluster, "instrument handle out"=w394:refnum<k15>)  [unwired: 6 in]
        n218 = call <instrlib>:"niDCPower Configure Output Enabled.vi"("error in (no error)"=w363, "output enabled"=w291, "channel name"="0", "instrument handle"=w366) -> ("error out"=w397:errorcluster, "instrument handle out"=w396:refnum<k15>)  [unwired: 6 in]
        n219 = call <instrlib>:"niDCPower Configure Output Enabled.vi"("error in (no error)"=w364, "output enabled"=w291, "channel name"="1", "instrument handle"=w365) -> ("error out"=w398:errorcluster, "instrument handle out"=w399:refnum<k15>)  [unwired: 6 in]
        n220 = call <instrlib>:"niDCPower Configure Output Enabled.vi"("error in (no error)"=w305, "output enabled"=w291, "channel name"="2", "instrument handle"=w304) -> ("error out"=w299:errorcluster, "instrument handle out"=w298:refnum<k15>)  [unwired: 6 in]
        n221 = call <instrlib>:"niDCPower Configure Output Enabled.vi"("error in (no error)"=w341, "output enabled"=w291, "channel name"="0", "instrument handle"=w344) -> ("error out"=w384:errorcluster, "instrument handle out"=w383:refnum<k15>)  [unwired: 6 in]
        n222 = call <instrlib>:"niDCPower Configure Output Enabled.vi"("error in (no error)"=w342, "output enabled"=w291, "channel name"="1", "instrument handle"=w343) -> ("error out"=w385:errorcluster, "instrument handle out"=w386:refnum<k15>)  [unwired: 6 in]
        n223 = call <instrlib>:"niDCPower Configure Output Enabled.vi"("error in (no error)"=w331, "output enabled"=w291, "channel name"="0", "instrument handle"=w332) -> ("error out"=w323:errorcluster, "instrument handle out"=w324:refnum<k15>)  [unwired: 6 in]
        n224 = call <instrlib>:"niDCPower Configure Output Enabled.vi"("error in (no error)"=w319, "output enabled"=w291, "channel name"="2", "instrument handle"=w318) -> ("error out"=w314:errorcluster, "instrument handle out"=w313:refnum<k15>)  [unwired: 6 in]
        n225 = call <instrlib>:"niDCPower Measure.vi"("error in (no error)"=w384, "measurement type"=w296, "channel name"="0", "instrument handle"=w383) -> ("measurement"=→"ADC_cur":dbl, "instrument handle out"=w336:refnum<k15>)  [unwired: 5 in, 1 out]
        n226 = call <instrlib>:"niDCPower Measure.vi"("error in (no error)"=w385, "measurement type"=w296, "channel name"="1", "instrument handle"=w386) -> ("measurement"=→"STAB_cur":dbl)  [unwired: 5 in, 2 out]
        n227 = call <instrlib>:"niDCPower Measure.vi"("error in (no error)"=w314, "measurement type"=w296, "channel name"="2", "instrument handle"=w313) -> ("measurement"=→"-15_cur":dbl)  [unwired: 5 in, 2 out]
        n228 = call <instrlib>:"niDCPower Measure.vi"("error in (no error)"=w400, "measurement type"=w296, "channel name"="1", "instrument handle"=w393) -> ("measurement"=→"RD_cur":dbl, "instrument handle out"=w335:refnum<k15>)  [unwired: 5 in, 1 out]
        n229 = call <instrlib>:"niDCPower Measure.vi"("error in (no error)"=w395, "measurement type"=w296, "channel name"="2", "instrument handle"=w394) -> ("measurement"=→"PH_LOW_cur":dbl)  [unwired: 5 in, 2 out]
        n230 = call <instrlib>:"niDCPower Measure.vi"("error in (no error)"=w323, "measurement type"=w296, "channel name"="0", "instrument handle"=w324) -> ("measurement"=→"4V_cur":dbl)  [unwired: 5 in, 2 out]
        n231 = call <instrlib>:"niDCPower Measure.vi"("error in (no error)"=w397, "measurement type"=w296, "channel name"="0", "instrument handle"=w396) -> ("measurement"=→"1V_cur":dbl, "instrument handle out"=w334:refnum<k15>)  [unwired: 5 in, 1 out]
        n232 = call <instrlib>:"niDCPower Measure.vi"("error in (no error)"=w398, "measurement type"=w296, "channel name"="1", "instrument handle"=w399) -> ("measurement"=→"VDD_cur":dbl)  [unwired: 5 in, 2 out]
        n233 = call <instrlib>:"niDCPower Measure.vi"("error in (no error)"=w299, "measurement type"=w296, "channel name"="2", "instrument handle"=w298) -> ("measurement"=→"PS_LOW_cur":dbl)  [unwired: 5 in, 2 out]
      }
    }
    n234 = Wait (ms)(milliseconds to wait=u32 1) -> ()  [unwired: 1 out]
  }
  n235 = while {
    tunnel: w10 -> [w418]
    shift-right: ["文韧 世男!"] -> _
    shift-left: FALSE ("文韧 世男!") -> [w414]
    tunnel: w9 -> [_]
    tunnel: [w409] -> w2
    stop <- w419 stop-if-true
    # "Запрос кадра"
    n236 = local read "Линейки"() -> (w417:bool)
    n237 = local read "Питание"() -> (w416:bool)
    n238 = Greater?(x="文韧 世男!", y=w414) -> (0:w410:bool)
    n239 = Or(x=w410, y="НЕПРЕРЫВНО") -> (x .or. y?=w412:bool)
    n240 = Compound Arithmetic op=AND(w412, w417, w416) -> (w415:bool)
    n241 = case shown="True" w415 {
      tunnel: w418 -> [w420 w423]
      tunnel: [w420 w422] -> w409
      frame False {
        n242 = Wait (ms)(milliseconds to wait=u32 1) -> ()  [unwired: 1 out]
      }
      frame True {
        n243 = stacked-sequence {
          seq-local: [_ w435 _ _ _ _] -> [_ _ w490 _ _ _]
          seq-local: [_ _ w500 _ _ _] -> [_ _ _ w522 _ _]
          seq-local: [_ _ _ w521 _ _] -> [_ _ _ _ w526 _]
          tunnel: w423 -> [w424 w436 _ _ _ _]
          tunnel: [_ w430 _ _ _ _] -> w422
          frame #0 {
            n244 = xnode "Invoke Method"("FPGA VI Reference In"=w424, "Number of Elements"=u32 0, "Timeout (ms)"=0) -> ("FPGA VI Reference Out"=w429:refnum<k20>, "Elements Remaining"=w428:u32)  [unwired: 1 in, 2 out]
            n245 = xnode "Invoke Method"("FPGA VI Reference In"=w429, "Number of Elements"=w428, "Timeout (ms)"=0) -> ()  [unwired: 1 in, 4 out]
          }
          frame #1 {
            n246 = for {
              N: "Усреднение" -> [_]
              tunnel: w436 -> [w445]
              shift-right: [w442] -> w433
              shift-left: u64[] array[125550 elements] -> [w443]
              tunnel: [w441] -> w430
              n247 = stacked-sequence {
                seq-local: [_ w450 _ _] -> [_ _ w463 _]
                tunnel: w445 -> [w447 w449 w457 _]
                tunnel: [_ _ w459 _] -> w444
                tunnel: [_ _ w456 _] -> w441
                frame #0 {
                  n248 = xnode "Read/Write Control"("FPGA VI Reference In"=w447, "Кадр в FIFO"=TRUE) -> ()  [unwired: 1 in, 2 out]
                  n249 = Wait (ms)(milliseconds to wait=u32 300) -> ()  [unwired: 1 out]
                }
                frame #1 {
                  n250 = xnode "Invoke Method"("FPGA VI Reference In"=w449, "Number of Elements"=u32 0, "Timeout (ms)"=0) -> ("FPGA VI Reference Out"=w452:refnum<k20>, "Elements Remaining"=w451:u32)  [unwired: 1 in, 2 out]
                  n251 = xnode "Invoke Method"("FPGA VI Reference In"=w452, "Number of Elements"=w451, "Timeout (ms)"=0) -> ("Data"=w450:u8[])  [unwired: 1 in, 3 out]
                }
                frame #2 {
                  # "L"
                  # "H"
                  n252 = Decimate 1D Array(w463) -> (w462:u8[], w461:u8[])
                  n253 = for {
                    N: 125550 -> [_]
                    tunnel: w462 -> [w473]
                    tunnel: w461 -> [w472]
                    tunnel: [w464] -> w459 mode=indexing
                    i -> [w471]
                    n254 = Index Array(array=w472, index=w471) -> (element=w469:u8)
                    n255 = Index Array(array=w473, index=w471) -> (element=w470:u8)
                    n256 = To Unsigned Word Integer(number=w469) -> (unsigned 16bit integer=w465:u16)
                    n257 = To Unsigned Word Integer(number=w470) -> (unsigned 16bit integer=w468:u16)
                    n258 = Multiply(x=w468, y=u16 256) -> (x*y=w466:u16)
                    n259 = Add(x=w466, y=w465) -> (x+y=w464:u16)
                  }
                  n260 = xnode "Read/Write Control"("FPGA VI Reference In"=w457, "Кадр в FIFO"=FALSE) -> ("FPGA VI Reference Out"=w456:refnum<k20>)  [unwired: 1 in, 1 out]
                }
                frame #3 {
                  n261 = Wait (ms)(milliseconds to wait=u32 300) -> ()  [unwired: 1 out]
                }
              }
              n262 = Add(x=w444, y=w443) -> (x+y=w442:u64[])
            }
            n263 = local write "FRAME_OK"(FALSE ("FRAME_OK")) -> ()
            n264 = for {
              tunnel: w433 -> [w440] mode=indexing
              tunnel: "Усреднение" -> [w439]
              tunnel: [w437] -> w435 mode=indexing
              n265 = Divide(x=w440, y=w439) -> (x/y=w438:dbl)
              n266 = To Unsigned Word Integer(number=w438) -> (unsigned 16bit integer=w437:u16)
            }
          }
          frame #2 {
            w495 = 5 ("length")
            w494 = 5 ("length")
            n267 = Multiply(x=w490, y="ISO") -> (x*y=w489:dbl[])
            n268 = To Unsigned Word Integer(number=w489) -> (unsigned 16bit integer=w488:u16[])
            n269 = for {
              N: 270 -> [_]
              tunnel: [w517] -> w475 mode=indexing
              shift-right: [w516] -> _
              shift-left: w488 -> [w520]
              n270 = Delete From Array(array=w520, length=465, index=0) -> (deleted portion=w517:u16[], array with subset deleted=w516:u16[])
            }
            "FRAME" <- w475
            n271 = for {
              tunnel: w475 -> [w512] mode=indexing
              tunnel: [w511] -> w500 mode=indexing
              n272 = for {
                N: 465 -> [_]
                tunnel: [w515] -> w511 mode=indexing
                tunnel: w512 -> [w514] mode=indexing
                n273 = Bundle(w514, w514, w514, w514) -> (w515:cluster{u16, u16, u16, u16})  [unwired: 1 in]
              }
            }
            "OUT" <- w500
            n274 = Multiply(x=w494, y=w495) -> (x*y=w479:i32)
            n275 = Array Subset(array=w475, index (row)=5 ("index"), length (row)=w494, index (col)=5 ("index"), length (col)=w495) -> (w497:u16[][])
            n276 = Array Subset(array=w475, index (row)=5 ("index"), length (row)=5 ("length"), index (col)=5 ("index"), length (col)=5 ("length")) -> (w486:u16[][])
            n277 = Reshape Array(w497, w479) -> (w498:u16[])
            n278 = Reshape Array(w486, w479) -> (w482:u16[])
            n279 = for {
              tunnel: w498 -> [w510] mode=indexing
              shift-right: [w508] -> w499
              shift-left: u64 0 -> [w509]
              n280 = Add(x=w510, y=w509) -> (x+y=w508:u64)
            }
            n281 = Divide(x=w499, y=w479) -> (x/y=w476:dbl)
            "Среднее" <- w476
            n282 = for {
              tunnel: w476 -> [w506]
              tunnel: w482 -> [w507] mode=indexing
              shift-right: [w502] -> w487
              shift-left: 0.0 -> [w504]
              n283 = Subtract(x=w507, y=w506) -> (x-y=w505:dbl)
              n284 = Square(x=w505) -> (x^2=w503:dbl)
              n285 = Add(x=w503, y=w504) -> (x+y=w502:dbl)
            }
            n286 = Divide(x=w487, y=w479) -> (x/y=w478:dbl)
            n287 = Square Root(x=w478) -> (sqrt(x)=→"СКО":dbl)
          }
          frame #3 {
            w523 = T5 6 items=["Grayscale (U8)", "Grayscale (I16)", "Grayscale (SGL)", "Complex (CSG)", "RGB (U32)", "HSL (U32)", "RGB (U64)"] ("Image Type")
            n288 = call "IMAQ Create"("Image Name"="FPZC", "Image Type"=w523) -> ("New Image"=w525:T1)  [unwired: 3 in, 1 out]
            n289 = call "IMAQ ArrayToColorImage"("Image"=w525, "Image Pixels (U64)"=w522) -> ("Image Out"=w521:T1)  [unwired: 3 in, 1 out]
            "Image" <- w521
          }
          frame #4 {
            n290 = case shown="True" "Запись Кадра" {
              tunnel: w526 -> [_ w531]
              frame False {
              }
              frame True {
                w536 = i16 0 ("precision (6)")
                w530 = "_"
                n291 = local read "Между кадрами, мс"() -> (w548:u8)
                n292 = local read "Номер образца"() -> (w542:string)
                n293 = Concatenate Strings("Образец_" ("string"), w542) -> (w537:string)
                n294 = Get Date/Time In Seconds() -> (seconds since 1Jan1904=w545:timestamp)
                n295 = Build Path(base path="Frames", name or relative path=w537) -> (appended path=w541:path)
                n296 = Number To Fractional String(number=w548, width (-)=w536, precision (6)=w536) -> (F-format string=w549:string)  [unwired: 1 in]
                n297 = Format Date/Time String(time format string (%c)="%H.%M.%S", seconds (now)=w545) -> (date/time string=w547:string)  [unwired: 1 in]
                n298 = call <vilib>:"Check if File or Folder Exists.vi"("path"=w541) -> ("file or folder exists?"=w540:bool, "dup path"=w539:path)  [unwired: 8 in, 1 out]
                n299 = case shown="False" w540 {
                  tunnel: w539 -> [w552 w553]
                  tunnel: [w551 w553] -> w546
                  frame False {
                    n300 = Create Folder(path (use dialog)=w552) -> (created path=w551:path)  [unwired: 2 in, 2 out]
                  }
                  frame True {
                  }
                }
                n301 = Concatenate Strings(w547, w530, "Тн=" ("string"), w549, "мс_" ("string"), "ПРИМЕЧАНИЕ", w530, "Какая фотка?", ".tiff" ("element")) -> (w543:string)
                n302 = Build Path(base path=w546, name or relative path=w543) -> (appended path=w544:path)
                n303 = call-poly "IMAQ Write File 2"("File Path"=w544, "Image"=w531) -> ()  [unwired: 8 in, 2 out]
              }
            }
          }
          frame #5 {
            "FRAME_OK" <- TRUE
          }
        }
      }
    }
    n304 = local read "Стоп"() -> (w419:bool)
  }
  n305 = while {
    tunnel: w10 -> [w561]
    shift-right: ["Прошить АЦП"] -> _
    shift-left: FALSE -> [w560]
    tunnel: w9 -> [_]
    tunnel: [w555] -> w4
    stop <- w562 stop-if-true
    n306 = Greater?(x="Прошить АЦП", y=w560) -> (0:w558:bool)
    n307 = local read "Питание"() -> (w556:bool)
    n308 = And(x=w556, y=w558) -> (x .and. y?=w557:bool)
    n309 = case shown="True" w557 {
      tunnel: w561 -> [w563 w566]
      tunnel: [w563 w565] -> w555
      frame False {
        n310 = Wait (ms)(milliseconds to wait=u32 1) -> ()  [unwired: 1 out]
      }
      frame True {
        n311 = stacked-sequence {
          tunnel: w566 -> [w592 w632 w646 w675 w719 w729 w754 w788 _]
          tunnel: [_ _ _ _ _ _ _ w779 _] -> w565
          frame #0 {
            w588 = TRUE ("element")
            w589 = FALSE
            # "8"
            # "0"
            # "Configuration"
            n312 = xnode "Read/Write Control"("FPGA VI Reference In"=w592, "Enum"=T6."Configuration") -> ("FPGA VI Reference Out"=w579:refnum<k20>)  [unwired: 1 in, 1 out]
            n313 = xnode "Read/Write Control"("FPGA VI Reference In"=w569, "Read(T)/Write(F)"=TRUE) -> ("FPGA VI Reference Out"=w575:refnum<k20>, "error out"=w574:errorcluster)  [unwired: 1 in]
            n314 = case shown="\"3CH\", Default" "3CH/1CH" {
              tunnel: [TRUE FALSE] -> w587
              frame "3CH", Default {
              }
              frame "1CH" {
              }
            }
            n315 = case shown="\"4V\"" "2/4 V" {
              tunnel: [FALSE TRUE] -> w585
              frame "2V", Default {
              }
              frame "4V" {
              }
            }
            n316 = xnode "Read/Write Control"("FPGA VI Reference In"=w579, "Read(T)/Write(F)"=FALSE) -> ("FPGA VI Reference Out"=w577:refnum<k20>)  [unwired: 1 in, 1 out]
            n317 = flat-sequence {
              tunnel: w575 -> [w604]
              tunnel: w574 -> [w603]
              tunnel: [w602] -> w573
              tunnel: [w601] -> w572
              frame #0 {
                n318 = xnode "Read/Write Control"("FPGA VI Reference In"=w604, "error in"=w603, "Конфигурация"=TRUE) -> ("FPGA VI Reference Out"=w602:refnum<k20>, "error out"=w601:errorcluster)
                n319 = Wait (ms)(milliseconds to wait=u32 10) -> ()  [unwired: 1 out]
              }
            }
            n320 = Build Array(w589, w589, w589, w588, w588, w587, w588, w585, FALSE) -> (w590:bool[])
            n321 = Reverse 1D Array(array=w590) -> (reversed array=w582:bool[])
            n322 = xnode "Read/Write Control"("FPGA VI Reference In"=w577, "Write Data"=w582) -> ("FPGA VI Reference Out"=w581:refnum<k20>)  [unwired: 1 in, 1 out]
            n323 = flat-sequence {
              tunnel: w573 -> [w598]
              tunnel: w572 -> [w597]
              tunnel: [w595] -> w571
              tunnel: [w594] -> w570
              frame #0 {
                n324 = xnode "Read/Write Control"("FPGA VI Reference In"=w598, "error in"=w597, "Конфигурация"=FALSE) -> ("FPGA VI Reference Out"=w595:refnum<k20>, "error out"=w594:errorcluster)
                n325 = Wait (ms)(milliseconds to wait=u32 10) -> ()  [unwired: 1 out]
              }
            }
            n326 = flat-sequence {
              tunnel: w581 -> [w612]
              tunnel: [w610] -> w580
              frame #0 {
                n327 = xnode "Read/Write Control"("FPGA VI Reference In"=w612, "Конфигурация"=TRUE) -> ("FPGA VI Reference Out"=w610:refnum<k20>)  [unwired: 1 in, 1 out]
                n328 = Wait (ms)(milliseconds to wait=u32 10) -> ()  [unwired: 1 out]
              }
            }
            n329 = local write "АЦП прошит!"(FALSE ("АЦП прошит!")) -> ()
            n330 = xnode "Read/Write Control"("FPGA VI Reference In"=w571, "error in"=w570) -> ("READ"=→"Configuration":bool[])  [unwired: 2 out]
            n331 = flat-sequence {
              tunnel: w580 -> [w608]
              tunnel: [w606] -> w569
              frame #0 {
                n332 = xnode "Read/Write Control"("FPGA VI Reference In"=w608, "Конфигурация"=FALSE) -> ("FPGA VI Reference Out"=w606:refnum<k20>)  [unwired: 1 in, 1 out]
                n333 = Wait (ms)(milliseconds to wait=u32 10) -> ()  [unwired: 1 out]
              }
            }
          }
          frame #1 {
            # "GREEN_OFFSET"
            n334 = case shown="\"-\", Default" "+/- OUT1" {
              tunnel: [TRUE FALSE] -> w619
              frame "-", Default {
              }
              frame "+" {
              }
            }
            n335 = Quotient & Remainder(x="Смещение, до 300_OUT1", y=1.171875) -> (floor(x/y)=w624:dbl)  [unwired: 1 out]
            n336 = xnode "Read/Write Control"("FPGA VI Reference In"=w632, "Enum"=T6."GREEN OFF" ("OFFSET")) -> ("FPGA VI Reference Out"=w631:refnum<k20>, "error out"=w630:errorcluster)  [unwired: 1 in]
            n337 = Subtract(x=w624, y=1.0) -> (x-y=w621:dbl)
            n338 = To Unsigned Byte Integer(number=w621) -> (unsigned 8bit integer=w620:u8)
            n339 = xnode "Read/Write Control"("FPGA VI Reference In"=w631, "error in"=w630, "Read(T)/Write(F)"=FALSE) -> ("FPGA VI Reference Out"=w629:refnum<k20>)  [unwired: 1 out]
            n340 = Number To Boolean Array(number=w620) -> (Boolean array=w618:bool[])
            n341 = Reverse 1D Array(array=w618) -> (reversed array=w617:bool[])
            n342 = Build Array (concatenate)(w619, w617) -> (w622:bool[])
            n343 = xnode "Read/Write Control"("FPGA VI Reference In"=w629, "Write Data"=w622) -> ("FPGA VI Reference Out"=w634:refnum<k20>)  [unwired: 1 in, 1 out]
            n344 = flat-sequence {
              tunnel: w634 -> [w645]
              tunnel: [w643] -> w633
              frame #0 {
                n345 = xnode "Read/Write Control"("FPGA VI Reference In"=w645, "Конфигурация"=TRUE) -> ("FPGA VI Reference Out"=w643:refnum<k20>)  [unwired: 1 in, 1 out]
                n346 = Wait (ms)(milliseconds to wait=u32 10) -> ()  [unwired: 1 out]
              }
            }
            n347 = flat-sequence {
              tunnel: w633 -> [w641]
              tunnel: [w639] -> _
              frame #0 {
                n348 = xnode "Read/Write Control"("FPGA VI Reference In"=w641, "Конфигурация"=FALSE) -> ("FPGA VI Reference Out"=w639:refnum<k20>)  [unwired: 1 in, 1 out]
                n349 = Wait (ms)(milliseconds to wait=u32 10) -> ()  [unwired: 1 out]
              }
            }
          }
          frame #2 {
            # "RED_OFFSET"
            n350 = case shown="\"-\", Default" "+/- OUT4" {
              tunnel: [TRUE FALSE] -> w662
              frame "-", Default {
              }
              frame "+" {
              }
            }
            n351 = Quotient & Remainder(x="Смещение, до 300_OUT4", y=1.171875) -> (floor(x/y)=w657:dbl)  [unwired: 1 out]
            n352 = xnode "Read/Write Control"("FPGA VI Reference In"=w646, "Enum"=T6."RED OFF" ("OFFSET")) -> ("FPGA VI Reference Out"=w653:refnum<k20>, "error out"=w654:errorcluster)  [unwired: 1 in]
            n353 = Subtract(x=w657, y=1.0) -> (x-y=w660:dbl)
            n354 = To Unsigned Byte Integer(number=w660) -> (unsigned 8bit integer=w661:u8)
            n355 = xnode "Read/Write Control"("FPGA VI Reference In"=w653, "error in"=w654, "Read(T)/Write(F)"=FALSE) -> ("FPGA VI Reference Out"=w655:refnum<k20>)  [unwired: 1 out]
            n356 = Number To Boolean Array(number=w661) -> (Boolean array=w663:bool[])
            n357 = Reverse 1D Array(array=w663) -> (reversed array=w664:bool[])
            n358 = Build Array (concatenate)(w662, w664) -> (w659:bool[])
            n359 = xnode "Read/Write Control"("FPGA VI Reference In"=w655, "Write Data"=w659) -> ("FPGA VI Reference Out"=w651:refnum<k20>)  [unwired: 1 in, 1 out]
            n360 = flat-sequence {
              tunnel: w651 -> [w674]
              tunnel: [w672] -> w652
              frame #0 {
                n361 = xnode "Read/Write Control"("FPGA VI Reference In"=w674, "Конфигурация"=TRUE) -> ("FPGA VI Reference Out"=w672:refnum<k20>)  [unwired: 1 in, 1 out]
                n362 = Wait (ms)(milliseconds to wait=u32 10) -> ()  [unwired: 1 out]
              }
            }
            n363 = flat-sequence {
              tunnel: w652 -> [w670]
              tunnel: [w668] -> _
              frame #0 {
                n364 = xnode "Read/Write Control"("FPGA VI Reference In"=w670, "Конфигурация"=FALSE) -> ("FPGA VI Reference Out"=w668:refnum<k20>)  [unwired: 1 in, 1 out]
                n365 = Wait (ms)(milliseconds to wait=u32 10) -> ()  [unwired: 1 out]
              }
            }
          }
          frame #3 {
            # "BLUE_OFFSET"
            n366 = case shown="\"-\", Default" "+/- OUT2" {
              tunnel: [TRUE FALSE] -> w691
              frame "-", Default {
              }
              frame "+" {
              }
            }
            n367 = Quotient & Remainder(x="Смещение, до 300_OUT2", y=1.171875) -> (floor(x/y)=w686:dbl)  [unwired: 1 out]
            n368 = xnode "Read/Write Control"("FPGA VI Reference In"=w675, "Enum"=T6."BLUE OFF" ("OFFSET")) -> ("FPGA VI Reference Out"=w682:refnum<k20>, "error out"=w683:errorcluster)  [unwired: 1 in]
            n369 = Subtract(x=w686, y=1.0) -> (x-y=w689:dbl)
            n370 = To Unsigned Byte Integer(number=w689) -> (unsigned 8bit integer=w690:u8)
            n371 = xnode "Read/Write Control"("FPGA VI Reference In"=w682, "error in"=w683, "Read(T)/Write(F)"=FALSE) -> ("FPGA VI Reference Out"=w684:refnum<k20>)  [unwired: 1 out]
            n372 = Number To Boolean Array(number=w690) -> (Boolean array=w692:bool[])
            n373 = Reverse 1D Array(array=w692) -> (reversed array=w693:bool[])
            n374 = Build Array (concatenate)(w691, w693) -> (w688:bool[])
            n375 = xnode "Read/Write Control"("FPGA VI Reference In"=w684, "Write Data"=w688) -> ("FPGA VI Reference Out"=w680:refnum<k20>)  [unwired: 1 in, 1 out]
            n376 = flat-sequence {
              tunnel: w680 -> [w703]
              tunnel: [w701] -> w681
              frame #0 {
                n377 = xnode "Read/Write Control"("FPGA VI Reference In"=w703, "Конфигурация"=TRUE) -> ("FPGA VI Reference Out"=w701:refnum<k20>)  [unwired: 1 in, 1 out]
                n378 = Wait (ms)(milliseconds to wait=u32 10) -> ()  [unwired: 1 out]
              }
            }
            n379 = flat-sequence {
              tunnel: w681 -> [w699]
              tunnel: [w697] -> _
              frame #0 {
                n380 = xnode "Read/Write Control"("FPGA VI Reference In"=w699, "Конфигурация"=FALSE) -> ("FPGA VI Reference Out"=w697:refnum<k20>)  [unwired: 1 in, 1 out]
                n381 = Wait (ms)(milliseconds to wait=u32 10) -> ()  [unwired: 1 out]
              }
            }
          }
          frame #4 {
            w714 = FALSE
            # "GREEN PGA"
            n382 = Decrement(x="Усиление (до 6)_OUT1") -> (x-1=w706:u8)
            n383 = Multiply(x=w706, y=378) -> (x*y=w708:i32)
            n384 = Multiply(x="Усиление (до 6)_OUT1", y=5) -> (x*y=w711:i32)
            n385 = xnode "Read/Write Control"("FPGA VI Reference In"=w719, "Enum"=T6."GREEN PGA" ("PGA")) -> ("FPGA VI Reference Out"=w717:refnum<k20>)  [unwired: 1 in, 1 out]
            n386 = Divide(x=w708, y=w711) -> (x/y=w712:dbl)
            n387 = Number To Boolean Array(number=w712) -> (Boolean array=w705:bool[])
            n388 = xnode "Read/Write Control"("FPGA VI Reference In"=w717, "Read(T)/Write(F)"=FALSE) -> ("FPGA VI Reference Out"=w716:refnum<k20>)  [unwired: 1 in, 1 out]
            n389 = Build Array (concatenate)(w714, w714, w714, w705) -> (w713:bool[])
            n390 = xnode "Read/Write Control"("FPGA VI Reference In"=w716, "Write Data"=w713) -> ("FPGA VI Reference Out"=w718:refnum<k20>)  [unwired: 1 in, 1 out]
            n391 = flat-sequence {
              tunnel: [w727] -> w720
              tunnel: w718 -> [w726]
              frame #0 {
                n392 = xnode "Read/Write Control"("FPGA VI Reference In"=w726, "Конфигурация"=TRUE) -> ("FPGA VI Reference Out"=w727:refnum<k20>)  [unwired: 1 in, 1 out]
                n393 = Wait (ms)(milliseconds to wait=u32 10) -> ()  [unwired: 1 out]
              }
            }
            n394 = flat-sequence {
              tunnel: w720 -> [w724]
              tunnel: [w722] -> _
              frame #0 {
                n395 = xnode "Read/Write Control"("FPGA VI Reference In"=w724, "Конфигурация"=FALSE) -> ("FPGA VI Reference Out"=w722:refnum<k20>)  [unwired: 1 in, 1 out]
                n396 = Wait (ms)(milliseconds to wait=u32 10) -> ()  [unwired: 1 out]
              }
            }
          }
          frame #5 {
            w732 = FALSE
            # "BLUE PGA"
            n397 = Decrement(x="Усиление (до 6)_OUT2") -> (x-1=w736:u8)
            n398 = Multiply(x=w736, y=378) -> (x*y=w737:i32)
            n399 = Multiply(x="Усиление (до 6)_OUT2", y=5) -> (x*y=w739:i32)
            n400 = xnode "Read/Write Control"("FPGA VI Reference In"=w729, "Enum"=T6."BLUE PGA" ("PGA")) -> ("FPGA VI Reference Out"=w743:refnum<k20>)  [unwired: 1 in, 1 out]
            n401 = Divide(x=w737, y=w739) -> (x/y=w740:dbl)
            n402 = Number To Boolean Array(number=w740) -> (Boolean array=w735:bool[])
            n403 = xnode "Read/Write Control"("FPGA VI Reference In"=w743, "Read(T)/Write(F)"=FALSE) -> ("FPGA VI Reference Out"=w742:refnum<k20>)  [unwired: 1 in, 1 out]
            n404 = Build Array (concatenate)(w732, w732, w732, w735) -> (w741:bool[])
            n405 = xnode "Read/Write Control"("FPGA VI Reference In"=w742, "Write Data"=w741) -> ("FPGA VI Reference Out"=w744:refnum<k20>)  [unwired: 1 in, 1 out]
            n406 = flat-sequence {
              tunnel: [w752] -> w745
              tunnel: w744 -> [w751]
              frame #0 {
                n407 = xnode "Read/Write Control"("FPGA VI Reference In"=w751, "Конфигурация"=TRUE) -> ("FPGA VI Reference Out"=w752:refnum<k20>)  [unwired: 1 in, 1 out]
                n408 = Wait (ms)(milliseconds to wait=u32 10) -> ()  [unwired: 1 out]
              }
            }
            n409 = flat-sequence {
              tunnel: w745 -> [w749]
              tunnel: [w747] -> _
              frame #0 {
                n410 = xnode "Read/Write Control"("FPGA VI Reference In"=w749, "Конфигурация"=FALSE) -> ("FPGA VI Reference Out"=w747:refnum<k20>)  [unwired: 1 in, 1 out]
                n411 = Wait (ms)(milliseconds to wait=u32 10) -> ()  [unwired: 1 out]
              }
            }
          }
          frame #6 {
            w765 = FALSE
            # "RED PGA"
            n412 = Decrement(x="Усиление (до 6)_OUT4") -> (x-1=w757:u8)
            n413 = Multiply(x=w757, y=378) -> (x*y=w759:i32)
            n414 = Multiply(x="Усиление (до 6)_OUT4", y=5) -> (x*y=w762:i32)
            n415 = xnode "Read/Write Control"("FPGA VI Reference In"=w754, "Enum"=T6."RED PGA" ("PGA")) -> ("FPGA VI Reference Out"=w768:refnum<k20>)  [unwired: 1 in, 1 out]
            n416 = Divide(x=w759, y=w762) -> (x/y=w763:dbl)
            n417 = Number To Boolean Array(number=w763) -> (Boolean array=w756:bool[])
            n418 = xnode "Read/Write Control"("FPGA VI Reference In"=w768, "Read(T)/Write(F)"=FALSE) -> ("FPGA VI Reference Out"=w767:refnum<k20>)  [unwired: 1 in, 1 out]
            n419 = Build Array (concatenate)(w765, w765, w765, w756) -> (w764:bool[])
            n420 = xnode "Read/Write Control"("FPGA VI Reference In"=w767, "Write Data"=w764) -> ("FPGA VI Reference Out"=w769:refnum<k20>)  [unwired: 1 in, 1 out]
            n421 = flat-sequence {
              tunnel: [w777] -> w770
              tunnel: w769 -> [w776]
              frame #0 {
                n422 = xnode "Read/Write Control"("FPGA VI Reference In"=w776, "Конфигурация"=TRUE) -> ("FPGA VI Reference Out"=w777:refnum<k20>)  [unwired: 1 in, 1 out]
                n423 = Wait (ms)(milliseconds to wait=u32 10) -> ()  [unwired: 1 out]
              }
            }
            n424 = flat-sequence {
              tunnel: w770 -> [w774]
              tunnel: [w772] -> _
              frame #0 {
                n425 = xnode "Read/Write Control"("FPGA VI Reference In"=w774, "Конфигурация"=FALSE) -> ("FPGA VI Reference Out"=w772:refnum<k20>)  [unwired: 1 in, 1 out]
                n426 = Wait (ms)(milliseconds to wait=u32 10) -> ()  [unwired: 1 out]
              }
            }
          }
          frame #7 {
            # "MUX"
            n427 = xnode "Read/Write Control"("FPGA VI Reference In"=w788, "Enum"=T6."MUX") -> ("FPGA VI Reference Out"=w782:refnum<k20>)  [unwired: 1 in, 1 out]
            n428 = case shown="\"OUT1\", Default" "Какой канал?" {
              tunnel: [bool[] [FALSE, TRUE, FALSE, TRUE, FALSE, FALSE, FALSE, FALSE, FALSE] ("MUX_register") bool[] [FALSE, TRUE, FALSE, FALSE, TRUE, FALSE, FALSE, FALSE, FALSE] ("MUX_register") bool[] [FALSE, TRUE, TRUE, FALSE, FALSE, FALSE, FALSE, FALSE, FALSE] ("MUX_register")] -> w780
              frame "OUT1", Default {
              }
              frame "OUT2" {
              }
              frame "OUT3" {
              }
            }
            n429 = xnode "Read/Write Control"("FPGA VI Reference In"=w782, "Read(T)/Write(F)"=FALSE) -> ("FPGA VI Reference Out"=w784:refnum<k20>)  [unwired: 1 in, 1 out]
            n430 = xnode "Read/Write Control"("FPGA VI Reference In"=w784, "Write Data"=w780) -> ("FPGA VI Reference Out"=w785:refnum<k20>)  [unwired: 1 in, 1 out]
            n431 = flat-sequence {
              tunnel: [w798] -> w786
              tunnel: w785 -> [w797]
              frame #0 {
                n432 = xnode "Read/Write Control"("FPGA VI Reference In"=w797, "Конфигурация"=TRUE) -> ("FPGA VI Reference Out"=w798:refnum<k20>)  [unwired: 1 in, 1 out]
                n433 = Wait (ms)(milliseconds to wait=u32 10) -> ()  [unwired: 1 out]
              }
            }
            n434 = flat-sequence {
              tunnel: w786 -> [w795]
              tunnel: [w793] -> w779
              frame #0 {
                n435 = xnode "Read/Write Control"("FPGA VI Reference In"=w795, "Конфигурация"=FALSE) -> ("FPGA VI Reference Out"=w793:refnum<k20>)  [unwired: 1 in, 1 out]
                n436 = Wait (ms)(milliseconds to wait=u32 10) -> ()  [unwired: 1 out]
              }
            }
          }
          frame #8 {
            "АЦП прошит!" <- TRUE ("АЦП прошит!")
          }
        }
      }
    }
    n437 = local read "Стоп"() -> (w562:bool)
  }
  n438 = while {
    tunnel: w10 -> [w834]
    tunnel: [w833] -> w3
    tunnel: w9 -> [_]
    stop <- w832 stop-if-true
    # "Общие настройки"
    n439 = local read "Питание"() -> (w836:bool)
    n440 = And(x="Линейки", y=w836) -> (x .and. y?=w830:bool)
    n441 = local read "Стоп"() -> (w831:bool)
    n442 = xnode "Read/Write Control"("FPGA VI Reference In"=w834, "Остановка основного цикла"=w831, "Линейки"=w830, "Сколько строк?"="Сколько строк?", "1163"="1163", "PS1_2"="PS1_2", "PS1_1"="PS1_1", "PS21_1"="PS21_1", "PS21_2"="PS21_2", "PS3_1"="PS3_1", "PS3_2"="PS3_2", "PS41_1"="PS41_1", "PS41_2"="PS41_2", "CDS1_2"="CDS1_2", "CDS1_1"="CDS1_1", "CDS2_2"="CDS2_2", "CDS2_1"="CDS2_1", "ADC_2"="ADC_2", "ADC_1"="ADC_1", "RG_2"="RG_2", "RG1"="RG1", "PH2_2"="PH2_2", "PH2_1"="PH2_1", "PH1_2"="PH1_2", "PH1_1"="PH1_1", "HOR"="HOR", "8"="8", "LOW"="LOW", "HIGH"="HIGH", "Между кадрами"="Между кадрами, мс", "LED"="LED") -> ("FPGA VI Reference Out"=w833:refnum<k20>)  [unwired: 1 in, 1 out]
    n443 = Wait (ms)(milliseconds to wait=u32 1) -> ()  [unwired: 1 out]
    n444 = local read "Стоп"() -> (w832:bool)
  }
  n445 = call <instrlib>:"niDCPower Close.vi"("instrument handle"=w15) -> ()  [unwired: 10 in, 1 out]
  n446 = call <instrlib>:"niDCPower Close.vi"("instrument handle"=w14) -> ()  [unwired: 10 in, 1 out]
  n447 = call <instrlib>:"niDCPower Close.vi"("instrument handle"=w13) -> ()  [unwired: 10 in, 1 out]
  n448 = flat-sequence {
    tunnel: w4 -> [w837]
    tunnel: w3 -> [_]
    tunnel: w2 -> [_]
    tunnel: w1 -> [_]
    frame #0 {
      n449 = xnode "Close FPGA VI Reference"("FPGA VI Reference In"=w837) -> ()  [unwired: 1 in, 1 out]
    }
  }
